vi "control panel.vi"() -> ()   [LabVIEW 2026]
uses:
  <vilib>/Instr/_visa.llb/VISA Configure Serial Port (Instr).vi
panel:
  out "read buffer":string
  out "Mist Sprayer":bool
  out "Cooling Fan":bool
  out "Pump Running":bool
  in  "Humidity Threshold":dbl(slide) scale=0.0..100.0
  in  "Temperature Threshold":dbl(slide) scale=0.0..50.0
  in  "Soil Moisture Threshold":dbl(slide) scale=0.0..1023.0
  out "Tank Full":bool
  out "Thermometer":dbl(slide) scale=0.0..50.0
  out "Humidity":dbl(knob) scale=0.0..100.0
  out "Soil Moisture":dbl(knob) scale=0.0..1023.0
  in  "stop":bool
  in  "Port":refnum<visa-resource-name>
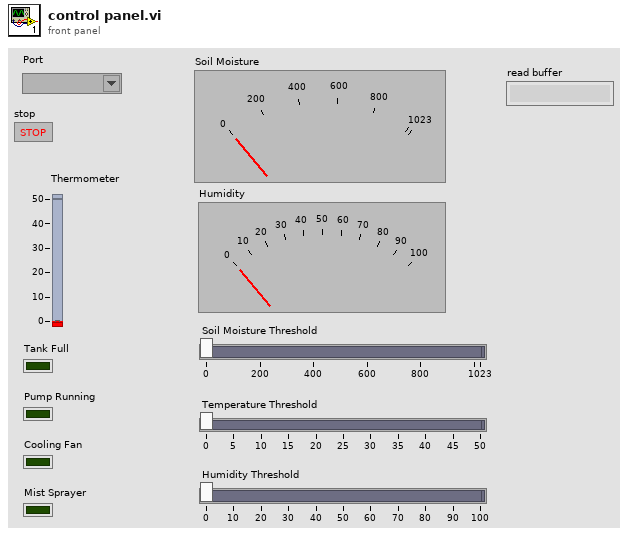
[diagram p1: front panel]
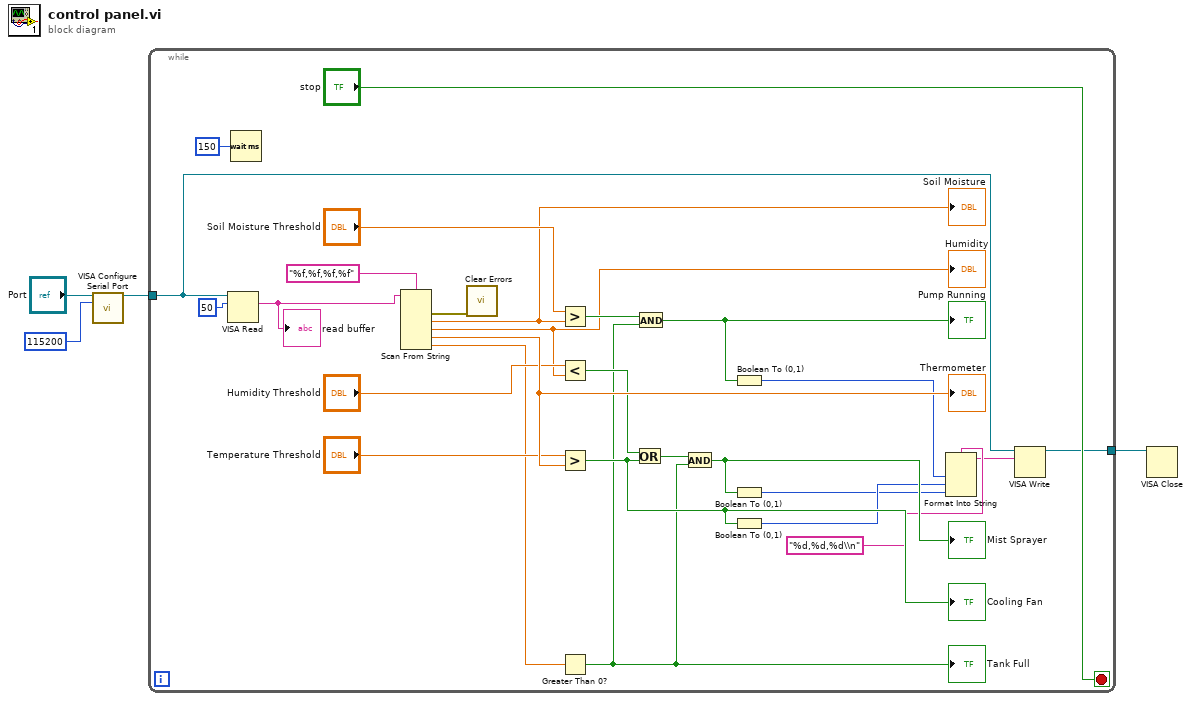
[diagram p0: block diagram]
diagram:
  n1 = call-poly "VISA Configure Serial Port"("VISA resource name"="Port", "baud rate (9600)"=u32 115200) -> ("VISA resource name out"=w2:refnum<visa-resource-name>)  [unwired: 12 in, 1 out]
  n2 = while {
    tunnel: w2 -> [w11]
    tunnel: [w10] -> w1
    stop <- "stop" stop-if-true
    n3 = VISA Read(VISA resource name=w11, byte count=u32 50) -> (read buffer=w7:string)  [unwired: 1 in, 3 out]
    "read buffer" <- w7
    n4 = Wait (ms)(milliseconds to wait=u32 150) -> ()  [unwired: 1 out]
    n5 = Scan From String(format string="%f,%f,%f,%f", input string=w7) -> (error out=w8:errorcluster, output 1=w26:dbl, output 2=w21:dbl, output 3=w24:dbl, output 4=w6:dbl)  [unwired: 6 in, 2 out]
    "Soil Moisture" <- w26
    "Humidity" <- w21
    "Thermometer" <- w24
    n6 = call <vilib>:"Clear Errors.vi"("error in (no error)"=w8) -> ()  [unwired: 5 in, 2 out]
    n7 = Greater?(x="Soil Moisture Threshold", y=w26) -> (0:w25:bool)
    n8 = Less?(x="Humidity Threshold", y=w21) -> (x < y?=w20:bool)
    n9 = Greater?(x="Temperature Threshold", y=w24) -> (0:w17:bool)
    "Cooling Fan" <- w17
    n10 = Greater Than 0?(x=w6) -> (x > 0?=w5:bool)
    "Tank Full" <- w5
    n11 = Or(x=w20, y=w17) -> (x .or. y?=w19:bool)
    n12 = And(x=w25, y=w5) -> (x .and. y?=w18:bool)
    "Pump Running" <- w18
    n13 = And(x=w19, y=w5) -> (x .and. y?=w16:bool)
    "Mist Sprayer" <- w16
    n14 = Boolean To (0,1)(Boolean=w18) -> (0, 1=w15:i16)
    n15 = Boolean To (0,1)(Boolean=w16) -> (0, 1=w13:i16)
    n16 = Boolean To (0,1)(Boolean=w17) -> (0, 1=w14:i16)
    n17 = Format Into String(format string="%d,%d,%d\\n", w15, w14, w13) -> (resulting string=w9:string)  [unwired: 2 in, 1 out]
    n18 = VISA Write(VISA resource name=w11, write buffer=w9) -> (VISA resource name out=w10:refnum<visa-resource-name>)  [unwired: 1 in, 2 out]
  }
  n19 = VISA Close(VISA resource name=w1) -> ()  [unwired: 1 in, 1 out]
